vi "RemoteVI Index HTML.vi"(11 "error in":errorcluster) -> (4 "html":string, 15 "error out":errorcluster)   [LabVIEW 2020, in "RemoteVI.lvlib"]
doc: "Returns the browser client, web\\index.html, as one string constant (45029 bytes, SHA-256 bd4df0f21e4f24879766d9c2ba5b297a308cdc7323f2ba91d4f2f1fba401afc3). Generated by scripts\\gen-index-html-vi.mjs - do not edit the constant by hand; regenerate it when the client changes. error in passes through unchanged."
uses:
  RemoteVI.lvlib
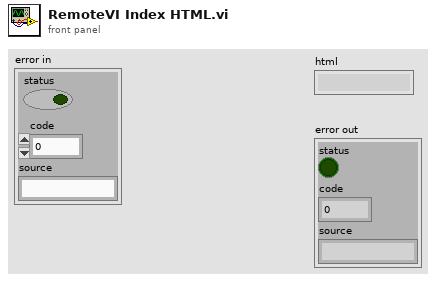
[diagram p1: front panel]
diagram:
  # "Generated from web/index.html"
  "html" <- "<!doctype html>\r\n<html lang=\"en\">\r\n<head>\r\n<meta charset=\"utf-8\">\r\n<meta name=\"viewport\" content=\"width=device-width, initial-scale=1, viewport-fit=cover\">\r\n<title>RemoteVI</title>\r\n<!--\r\n  RemoteVI browser client, protocol v2 (docs/protocol.md).\r\n  Self-contained on purpose: the LabVIEW toolkit embeds this one file as a string\r\n  constant and serves it for GET /, so a built EXE needs no support files.\r\n  Keep it pure ASCII (use \\u escapes and HTML entities) so the G string constant\r\n  holds exactly these bytes. After editing, regenerate the embedded copy:\r\n  node scripts/gen-index-html-vi.mjs --compose\r\n-->\r\n<style>\r\n:root {\r\n  --bg: #e9ebee; --bar-bg: #fff; --bar-fg: #1d2330; --muted: #667085;\r\n  --accent: #1f6feb; --ok: #1a7f37; --warn: #bf8700; --err: #cf222e; --border: #d0d7de;\r\n  --btn-hover: rgb(0 0 0 / 0.06);\r\n  color-scheme: light dark;\r\n}\r\n@media (prefers-color-scheme: dark) {\r\n  :root { --bg: #15181e; --bar-bg: #1e232b; --bar-fg: #e6edf3; --muted: #8d96a0; --border: #30363d; --btn-hover: rgb(255 255 255 / 0.08); }\r\n}\r\n* { box-sizing: border-box; }\r\nhtml, body { height: 100%; margin: 0; }\r\nbody {\r\n  display: flex; flex-direction: column; background: var(--bg); color: var(--bar-fg);\r\n  font: 13px/1.4 system-ui, -apple-system, \"Segoe UI\", sans-serif;\r\n}\r\n.bar {\r\n  display: flex; align-items: center; gap: 8px; padding: 6px 12px;\r\n  padding-left: max(12px, env(safe-area-inset-left)); padding-right: max(12px, env(safe-area-inset-right));\r\n  background: var(--bar-bg); border-bottom: 1px solid var(--border); flex-wrap: nowrap; min-height: 40px;\r\n}\r\n.title { display: flex; align-items: center; gap: 8px; min-width: 0; }\r\n.title strong { white-space: nowrap; overflow: hidden; text-overflow: ellipsis; }\r\n#status { color: var(--muted); white-space: nowrap; }\r\n.spacer { flex: 1; }\r\n.stats { color: var(--muted); font-variant-numeric: tabular-nums; white-space: nowrap; }\r\n.group { display: inline-flex; border: 1px solid var(--border); border-radius: 6px; overflow: hidden; }\r\n.group button + button { border-left: 1px solid var(--border); }\r\n.bar button {\r\n  font: inherit; min-width: 32px; height: 28px; padding: 0 9px; border: 0; background: transparent;\r\n  color: inherit; cursor: pointer; white-space: nowrap;\r\n}\r\n.bar > button { border: 1px solid var(--border); border-radius: 6px; }\r\n.bar button:hover { background: var(--btn-hover); }\r\n.bar button[aria-pressed=\"true\"] { color: var(--accent); background: color-mix(in srgb, var(--accent) 12%, transparent); }\r\n#zoom-label { min-width: 48px; text-align: center; color: var(--muted); font-variant-numeric: tabular-nums; }\r\n.dot { width: 9px; height: 9px; flex: none; border-radius: 50%; background: var(--warn); }\r\nbody[data-state=\"online\"] .dot { background: var(--ok); }\r\nbody[data-state=\"offline\"] .dot { background: var(--err); }\r\n#kbd-btn { display: none; }\r\nbody[data-touch=\"true\"] #kbd-btn { display: inline-block; }\r\n\r\n/* The stage scrolls; the wrapper is sized to the scaled frame so scrollbars match. */\r\n.stage { flex: 1; overflow: auto; padding: 16px; overscroll-behavior: contain; }\r\n.panel-wrap {\r\n  position: relative; margin: 0 auto; box-shadow: 0 1px 6px rgb(0 0 0 / 0.25);\r\n  touch-action: none; transform-origin: 0 0;\r\n}\r\n#panel { display: block; outline: none; cursor: default; touch-action: none; }\r\n#panel.pixelated { image-rendering: pixelated; }\r\nbody[data-view-only=\"true\"] #panel { cursor: not-allowed; }\r\n/* LabVIEW popups (menus, dropdowns, palette popups); may extend past the panel. */\r\n#overlay { position: absolute; left: 0; top: 0; transform-origin: 0 0; pointer-events: none; }\r\n#overlay img { position: absolute; display: block; pointer-events: auto; box-shadow: 2px 2px 6px rgb(0 0 0 / 0.35); }\r\n#overlay.pixelated img { image-rendering: pixelated; }\r\n/* Other windows of the application (dialogs, file dialogs, subVI panels). */\r\n#windows { position: absolute; left: 0; top: 0; width: 0; height: 0; }\r\n.win {\r\n  position: absolute; display: flex; flex-direction: column; background: var(--bar-bg);\r\n  border: 1px solid var(--border); border-radius: 8px; overflow: hidden;\r\n  box-shadow: 0 8px 28px rgb(0 0 0 / 0.35), 0 1px 4px rgb(0 0 0 / 0.2);\r\n}\r\n.win.active { border-color: var(--accent); }\r\n.win-title {\r\n  display: flex; align-items: center; gap: 8px; height: 30px; padding: 0 6px 0 10px; flex: none;\r\n  font-weight: 600; cursor: move; user-select: none; touch-action: none; border-bottom: 1px solid var(--border);\r\n}\r\n.win.active .win-title { background: color-mix(in srgb, var(--accent) 10%, var(--bar-bg)); }\r\n.win-title span { flex: 1; overflow: hidden; text-overflow: ellipsis; white-space: nowrap; }\r\n.win-title button {\r\n  width: 26px; height: 22px; border: 0; border-radius: 4px; background: transparent; color: inherit; font: inherit; cursor: pointer;\r\n}\r\n.win-title button:hover { background: var(--err); color: #fff; }\r\n.win canvas { display: block; touch-action: none; }\r\n.win canvas.pixelated { image-rendering: pixelated; }\r\n/* While a modal window is up the panel is disabled, as on the host. */\r\n#dim { position: absolute; inset: 0; background: rgb(0 0 0 / 0.28); display: none; }\r\n.panel-wrap.modal #dim { display: block; }\r\n#win-list { max-width: 180px; height: 28px; font: inherit; border: 1px solid var(--border); border-radius: 6px; background: var(--bar-bg); color: inherit; }\r\n#win-list[hidden] { display: none; }\r\n/* Tip strip of the control under the pointer, drawn like LabVIEW's own (tips message). */\r\n#tip {\r\n  position: fixed; z-index: 1000; display: none; max-width: 400px; padding: 2px 5px;\r\n  background: #ffffe1; color: #000; border: 1px solid #767676; box-shadow: 1px 2px 4px rgb(0 0 0 / 0.3);\r\n  font: 12px/1.35 \"Segoe UI\", Tahoma, sans-serif; white-space: pre-wrap; pointer-events: none;\r\n}\r\n#tip.show { display: block; }\r\n/* Splitter bars (splitters message): the client drags them itself and shows this line meanwhile. */\r\n#ghost { position: absolute; display: none; pointer-events: none; background: rgb(0 0 0 / 0.45); outline: 1px dashed #fff; }\r\n#ghost.show { display: block; }\r\n.panel-wrap.split-v, .panel-wrap.split-v #panel { cursor: col-resize; }\r\n.panel-wrap.split-h, .panel-wrap.split-h #panel { cursor: row-resize; }\r\n/* Hidden input that brings up the on-screen keyboard on touch devices. */\r\n#kbd { position: fixed; left: 0; bottom: 0; width: 1px; height: 1px; opacity: 0; border: 0; padding: 0; font-size: 16px; }\r\n.toast {\r\n  position: fixed; left: 50%; bottom: 24px; transform: translateX(-50%); padding: 6px 12px; border-radius: 6px;\r\n  background: rgb(0 0 0 / 0.75); color: #fff; font-size: 12px; pointer-events: none; opacity: 0; transition: opacity 0.3s;\r\n}\r\n.toast.show { opacity: 1; }\r\n@media (max-width: 720px) {\r\n  .stats, #status, #zoom-label { display: none; }\r\n  .bar { gap: 6px; padding-top: 4px; padding-bottom: 4px; }\r\n  .stage { padding: 8px; }\r\n}\r\n</style>\r\n</head>\r\n<body data-state=\"connecting\" data-touch=\"false\">\r\n<header class=\"bar\">\r\n  <span class=\"title\"><span class=\"dot\" aria-hidden=\"true\"></span><strong id=\"vi-name\">RemoteVI</strong></span>\r\n  <span id=\"status\" role=\"status\">Connecting&hellip;</span>\r\n  <span class=\"spacer\"></span>\r\n  <span id=\"stats\" class=\"stats\"></span>\r\n  <span class=\"group\" role=\"group\" aria-label=\"Scaling\">\r\n    <button type=\"button\" data-mode=\"actual\" title=\"Actual size: one LabVIEW pixel per screen pixel (1)\">1:1</button>\r\n    <button type=\"button\" data-mode=\"fit\" title=\"Fit the whole window into the view (F)\">Fit</button>\r\n    <button type=\"button\" data-mode=\"width\" title=\"Fit the width, scroll vertically (W)\">Width</button>\r\n  </span>\r\n  <span class=\"group\" role=\"group\" aria-label=\"Zoom\">\r\n    <button type=\"button\" id=\"zoom-out\" title=\"Zoom out (-)\">&minus;</button>\r\n    <button type=\"button\" id=\"zoom-label\" title=\"Back to actual size\">100%</button>\r\n    <button type=\"button\" id=\"zoom-in\" title=\"Zoom in (+)\">+</button>\r\n  </span>\r\n  <select id=\"win-list\" title=\"Open windows\" hidden></select>\r\n  <button type=\"button\" id=\"kbd-btn\" title=\"Show the on-screen keyboard\">&#x2328;</button>\r\n  <button type=\"button\" id=\"fs-btn\" title=\"Fullscreen\">&#x26F6;</button>\r\n</header>\r\n<main id=\"stage\" class=\"stage\">\r\n  <div class=\"panel-wrap\" id=\"wrap\">\r\n    <canvas id=\"panel\" tabindex=\"0\" width=\"1\" height=\"1\" aria-label=\"Remote front panel\"></canvas>\r\n    <div id=\"dim\"></div>\r\n    <div id=\"windows\"></div>\r\n    <div id=\"overlay\"></div>\r\n    <div id=\"ghost\"></div>\r\n  </div>\r\n</main>\r\n<input id=\"kbd\" type=\"text\" autocomplete=\"off\" autocapitalize=\"off\" autocorrect=\"off\" spellcheck=\"false\" aria-label=\"Keyboard input\">\r\n<div id=\"toast\" class=\"toast\" role=\"status\"></div>\r\n<div id=\"tip\" role=\"tooltip\"></div>\r\n<script>\r\n'use strict';\r\n\r\n// --- protocol v2 constants (docs/protocol.md) --------------------------------\r\n\r\nconst FRAME_MAGIC = 0x52;          // 'R'\r\nconst MSG_FRAME = 1;\r\nconst MSG_OVERLAY = 2;\r\nconst MSG_WINDOW_FRAME = 3;\r\nconst OVERLAY_HEADER = 4;          // magic, type, count u16\r\nconst WINDOW_FRAME_HEADER = 16;    // magic, type, id u32, seq u32, width u16, height u16, count u16\r\nconst WIN_TITLE_H = 31;            // CSS px of a window's title bar (+ border)\r\nconst FRAME_HEADER = 12;           // magic, type, seq u32, width u16, height u16, count u16\r\nconst RECT_HEADER = 8;             // x i16, y i16, length u32\r\n\r\n// Win32 message numbers. The server posts them to the panel window, so these\r\n// values ARE the protocol.\r\nconst WM = {\r\n  KEYDOWN: 0x0100, KEYUP: 0x0101, CHAR: 0x0102,\r\n  MOUSEMOVE: 0x0200,\r\n  LBUTTONDOWN: 0x0201, LBUTTONUP: 0x0202, LBUTTONDBLCLK: 0x0203,\r\n  RBUTTONDOWN: 0x0204, RBUTTONUP: 0x0205, RBUTTONDBLCLK: 0x0206,\r\n  MBUTTONDOWN: 0x0207, MBUTTONUP: 0x0208, MBUTTONDBLCLK: 0x0209,\r\n  MOUSEWHEEL: 0x020A,\r\n};\r\nconst MK = { LBUTTON: 0x01, RBUTTON: 0x02, SHIFT: 0x04, CONTROL: 0x08, MBUTTON: 0x10 };\r\nconst WHEEL_DELTA = 120;\r\n\r\n// Browser button index (0 left, 1 middle, 2 right) -> [down, up, dblclk].\r\nconst BUTTON_MSGS = {\r\n  0: [WM.LBUTTONDOWN, WM.LBUTTONUP, WM.LBUTTONDBLCLK],\r\n  1: [WM.MBUTTONDOWN, WM.MBUTTONUP, WM.MBUTTONDBLCLK],\r\n  2: [WM.RBUTTONDOWN, WM.RBUTTONUP, WM.RBUTTONDBLCLK],\r\n};\r\n\r\n// KeyboardEvent.code -> [virtual-key code, extended-key flag]. Printable\r\n// characters are not listed: they travel as WM_CHAR so the remote side does not\r\n// depend on the host's keyboard layout.\r\nconst VK = {\r\n  Backspace: [0x08, 0], Tab: [0x09, 0], Enter: [0x0D, 0], NumpadEnter: [0x0D, 1],\r\n  ShiftLeft: [0x10, 0], ShiftRight: [0x10, 0], ControlLeft: [0x11, 0], ControlRight: [0x11, 1],\r\n  Escape: [0x1B, 0], PageUp: [0x21, 1], PageDown: [0x22, 1], End: [0x23, 1], Home: [0x24, 1],\r\n  ArrowLeft: [0x25, 1], ArrowUp: [0x26, 1], ArrowRight: [0x27, 1], ArrowDown: [0x28, 1],\r\n  Insert: [0x2D, 1], Delete: [0x2E, 1],\r\n  F1: [0x70, 0], F2: [0x71, 0], F3: [0x72, 0], F4: [0x73, 0], F5: [0x74, 0], F6: [0x75, 0],\r\n  F7: [0x76, 0], F8: [0x77, 0], F9: [0x78, 0], F10: [0x79, 0], F11: [0x7A, 0], F12: [0x7B, 0],\r\n};\r\n\r\nconst ZOOM_STEPS = [0.25, 0.33, 0.5, 0.67, 0.75, 0.9, 1, 1.25, 1.5, 2, 2.5, 3, 4];\r\nconst ZOOM_MIN = 0.1;\r\nconst ZOOM_MAX = 4;\r\nconst LONG_PRESS_MS = 550;      // touch: hold this long without moving = right click\r\nconst TAP_SLOP_PX = 8;          // touch: moving further than this starts a drag\r\nconst TIP_DELAY_MS = 500;       // hover this long on a control to see its tip strip\r\n\r\nfunction mouseFlags(e) {\r\n  let w = 0;\r\n  if (e.buttons & 1) w |= MK.LBUTTON;\r\n  if (e.buttons & 2) w |= MK.RBUTTON;\r\n  if (e.buttons & 4) w |= MK.MBUTTON;\r\n  if (e.shiftKey) w |= MK.SHIFT;\r\n  if (e.ctrlKey) w |= MK.CONTROL;\r\n  return w;\r\n}\r\n\r\n// lParam for WM_KEYDOWN / WM_KEYUP: repeat count 1, extended bit 24, and for\r\n// key-up the previous-state and transition bits. Sent as an unsigned decimal.\r\nfunction keyLParam(extended, up) {\r\n  let l = 1;\r\n  if (extended) l += 0x01000000;\r\n  if (up) l += 0xC0000000;\r\n  return l;\r\n}\r\n\r\nfunction readRects(v, buf, o, count) {\r\n  const rects = [];\r\n  for (let i = 0; i < count; i++) {\r\n    if (o + RECT_HEADER > buf.byteLength) throw new Error('truncated message');\r\n    const x = v.getInt16(o), y = v.getInt16(o + 2), len = v.getUint32(o + 4);\r\n    o += RECT_HEADER;\r\n    if (o + len > buf.byteLength) throw new Error('truncated message');\r\n    rects.push({ x, y, png: new Blob([new Uint8Array(buf, o, len)], { type: 'image/png' }) });\r\n    o += len;\r\n  }\r\n  return rects;\r\n}\r\n\r\nfunction decodeOverlay(buf) {\r\n  const v = new DataView(buf);\r\n  return readRects(v, buf, OVERLAY_HEADER, v.getUint16(2));\r\n}\r\n\r\nfunction decodeWindowFrame(buf) {\r\n  const v = new DataView(buf);\r\n  if (buf.byteLength < WINDOW_FRAME_HEADER) throw new Error('truncated window frame');\r\n  return {\r\n    id: v.getUint32(2), seq: v.getUint32(6), width: v.getUint16(10), height: v.getUint16(12),\r\n    rects: readRects(v, buf, WINDOW_FRAME_HEADER, v.getUint16(14)),\r\n  };\r\n}\r\n\r\nfunction decodeFrame(buf) {\r\n  const v = new DataView(buf);\r\n  if (buf.byteLength < FRAME_HEADER || v.getUint8(0) !== FRAME_MAGIC || v.getUint8(1) !== MSG_FRAME) {\r\n    throw new Error('not a RemoteVI frame');\r\n  }\r\n  return {\r\n    seq: v.getUint32(2), width: v.getUint16(6), height: v.getUint16(8),\r\n    rects: readRects(v, buf, FRAME_HEADER, v.getUint16(10)),\r\n  };\r\n}\r\n\r\n// Per-viewer preference; storage can be unavailable (private mode, blocked site data).\r\nconst prefs = {\r\n  get(key, fallback) {\r\n    try { return localStorage.getItem(`remotevi.${key}`) ?? fallback; } catch { return fallback; }\r\n  },\r\n  set(key, value) {\r\n    try { localStorage.setItem(`remotevi.${key}`, value); } catch { /* not persisted */ }\r\n  },\r\n};\r\n\r\n// --- client -------------------------------------------------------------------\r\n\r\nclass RemoteViClient {\r\n  constructor() {\r\n    this.canvas = document.getElementById('panel');\r\n    this.wrap = document.getElementById('wrap');\r\n    this.overlay = document.getElementById('overlay');\r\n    this.ctx = this.canvas.getContext('2d', { alpha: false });\r\n    this.stage = document.getElementById('stage');\r\n    this.statusEl = document.getElementById('status');\r\n    this.statsEl = document.getElementById('stats');\r\n    this.kbd = document.getElementById('kbd');\r\n    this.ws = null;\r\n    this.backoff = 250;\r\n    this.queue = Promise.resolve();   // frames are painted strictly in order\r\n    this.pendingMove = null;\r\n    this.stats = { frames: 0, bytes: 0, since: performance.now() };\r\n    this.origin = { x: 0, y: 0 };     // where the panel starts inside the frame\r\n    this.touches = new Map();         // pointerId -> {x, y} for touch gestures\r\n    this.touch = null;                // single-finger state (tap / long press / drag)\r\n    this.pinch = null;                // two-finger state\r\n    this.windows = new Map();         // id -> {info, el, canvas, ctx, dx, dy} (docs/protocol.md 7)\r\n    this.windowsLayer = document.getElementById('windows');\r\n    this.winList = document.getElementById('win-list');\r\n    this.pressWin = null;             // window a mouse press started in (keeps a drag on it)\r\n    this.tips = [];                   // tip strips {x, y, w, h, text} in frame coordinates (tips message)\r\n    this.tipEl = document.getElementById('tip');\r\n    this.tip = { at: null, timer: 0, quiet: null };  // control hovered, dwell timer, tip silenced by a click\r\n    this.splitters = [];              // draggable splitter bars {id, x, y, w, h, vertical, min, max} (splitters message)\r\n    this.split = null;                // splitter drag in progress {bar, pos, pointerId}\r\n    this.ghost = document.getElementById('ghost');\r\n\r\n    const coarse = matchMedia('(pointer: coarse)').matches;\r\n    document.body.dataset.touch = String(coarse);\r\n    this.mode = prefs.get('mode', coarse ? 'width' : 'actual');\r\n    this.zoom = Number(prefs.get('zoom', '1')) || 1;\r\n\r\n    this.bindView();\r\n    this.bindInput();\r\n    this.bindKeyboard();\r\n    this.winList.addEventListener('change', () => {\r\n      const w = this.windows.get(Number(this.winList.value));\r\n      if (w) { this.raise(w); w.el.scrollIntoView({ block: 'nearest', inline: 'nearest' }); }\r\n    });\r\n    setInterval(() => this.showStats(), 1000);\r\n    this.applyView();\r\n    this.connect();\r\n  }\r\n\r\n  // --- connection ----------------------------------------------------------------\r\n\r\n  connect() {\r\n    const scheme = location.protocol === 'https:' ? 'wss' : 'ws';\r\n    // The share's access token travels in the page URL (?t=...) and is required for the WebSocket too.\r\n    const token = new URLSearchParams(location.search).get('t') ?? '';\r\n    const ws = new WebSocket(`${scheme}://${location.host}/ws?t=${encodeURIComponent(token)}`);\r\n    ws.binaryType = 'arraybuffer';\r\n    this.ws = ws;\r\n    this.setStatus('connecting', 'Connecting...');\r\n    let opened = false;\r\n    ws.onopen = () => { opened = true; this.backoff = 250; this.setStatus('online', 'Connected'); };\r\n    ws.onmessage = (ev) => {\r\n      if (typeof ev.data === 'string') this.onText(ev.data);\r\n      else this.onFrame(ev.data);\r\n    };\r\n    ws.onclose = () => {\r\n      if (this.ws !== ws) return;\r\n      const retry = `retrying in ${(this.backoff / 1000).toFixed(1)} s`;\r\n      // The server answers a missing or wrong token with 403, which a browser reports as a plain close.\r\n      const why = opened ? 'Disconnected'\r\n        : !token ? 'This link has no access token (?t=...): open the full link of the share'\r\n          : 'Not connected: the access token is wrong, or the share has stopped';\r\n      this.setStatus('offline', `${why}, ${retry}`);\r\n      setTimeout(() => this.connect(), this.backoff);\r\n      this.backoff = Math.min(this.backoff * 2, 5000);\r\n    };\r\n  }\r\n\r\n  send(line) {\r\n    if (this.ws?.readyState === WebSocket.OPEN) this.ws.send(line);\r\n  }\r\n\r\n  onText(text) {\r\n    // Server text messages (docs/protocol.md 3.3). Unknown ones are ignored.\r\n    const sp = text.indexOf(' ');\r\n    const cmd = sp < 0 ? text : text.slice(0, sp);\r\n    const arg = sp < 0 ? '' : text.slice(sp + 1);\r\n    if (cmd === 'title') {\r\n      document.getElementById('vi-name').textContent = arg;\r\n      document.title = `${arg} - RemoteVI`;\r\n    } else if (cmd === 'viewonly') {\r\n      document.body.dataset.viewOnly = String(arg === '1');\r\n    } else if (cmd === 'windows') {\r\n      let list;\r\n      try { list = JSON.parse(arg); } catch { return; }\r\n      if (Array.isArray(list)) this.updateWindows(list);\r\n    } else if (cmd === 'origin') {\r\n      const [x, y] = arg.split(' ').map(Number);\r\n      if (Number.isFinite(x) && Number.isFinite(y)) this.origin = { x, y };\r\n    } else if (cmd === 'tips') {\r\n      let list;\r\n      try { list = JSON.parse(arg); } catch { return; }\r\n      if (!Array.isArray(list)) return;\r\n      this.tips = list.filter((t) => t && typeof t.text === 'string'\r\n        && [t.x, t.y, t.w, t.h].every(Number.isFinite));\r\n      this.hideTip();\r\n    } else if (cmd === 'splitters') {\r\n      let list;\r\n      try { list = JSON.parse(arg); } catch { return; }\r\n      if (!Array.isArray(list)) return;\r\n      this.splitters = list.filter((b) => b && Number.isInteger(b.id)\r\n        && [b.x, b.y, b.w, b.h, b.min, b.max].every(Number.isFinite));\r\n    }\r\n  }\r\n\r\n  // --- splitter bars (docs/protocol.md 3.3, 4) ----------------------------------------\r\n  // LabVIEW moves a splitter bar only while it tracks the real mouse, so the client drags\r\n  // the bar itself (a line follows the pointer) and sends `s <id> <pos>` on release; the\r\n  // server sets the splitter's position through VI Server.\r\n\r\n  /** The draggable bar under a client point, or null (not over a popup, a window or while modal). */\r\n  splitterAt(clientX, clientY) {\r\n    if (!this.splitters.length || this.overlay.childElementCount || this.wrap.classList.contains('modal')\r\n        || this.windowAt(clientX, clientY)) return null;\r\n    const { x, y } = this.framePoint(clientX, clientY, null);\r\n    // A thin bar is easier to hit with a few pixels of slack across it.\r\n    return this.splitters.find((b) => {\r\n      const sx = b.vertical ? 3 : 0, sy = b.vertical ? 0 : 3;\r\n      return x >= b.x - sx && x < b.x + b.w + sx && y >= b.y - sy && y < b.y + b.h + sy;\r\n    }) ?? null;\r\n  }\r\n\r\n  /** Cursor hint over a bar. */\r\n  splitterHover(clientX, clientY) {\r\n    const b = this.split?.bar ?? this.splitterAt(clientX, clientY);\r\n    this.wrap.classList.toggle('split-v', !!b?.vertical);\r\n    this.wrap.classList.toggle('split-h', !!b && !b.vertical);\r\n  }\r\n\r\n  splitStart(bar, e) {\r\n    this.hideTip(true);\r\n    this.split = { bar, pos: bar.vertical ? bar.x : bar.y, pointerId: e.pointerId, moved: false };\r\n    this.wrap.setPointerCapture(e.pointerId);\r\n    this.splitMove(e);\r\n  }\r\n\r\n  splitMove(e) {\r\n    const s = this.split;\r\n    const b = s.bar;\r\n    const { x, y } = this.framePoint(e.clientX, e.clientY, null);\r\n    const at = Math.round((b.vertical ? x - b.w / 2 : y - b.h / 2));\r\n    const pos = Math.max(b.min, Math.min(b.max, at));\r\n    if (pos !== s.pos) s.moved = true;\r\n    s.pos = pos;\r\n    const z = this.zoom;\r\n    const g = this.ghost.style;\r\n    g.left = `${(b.vertical ? pos : b.x) * z}px`;\r\n    g.top = `${(b.vertical ? b.y : pos) * z}px`;\r\n    g.width = `${Math.max(2, b.w * z)}px`;\r\n    g.height = `${Math.max(2, b.h * z)}px`;\r\n    this.ghost.classList.add('show');\r\n  }\r\n\r\n  splitEnd(cancel) {\r\n    const s = this.split;\r\n    this.split = null;\r\n    this.ghost.classList.remove('show');\r\n    if (!s || cancel || !s.moved) return;\r\n    const b = s.bar;\r\n    this.send(`s ${b.id} ${s.pos}`);\r\n  }\r\n\r\n  // --- tip strips (docs/protocol.md 3.3) ----------------------------------------------\r\n  // LabVIEW shows tip strips only while it is the foreground application, so the\r\n  // server sends the texts and the client shows them itself after a hover dwell.\r\n\r\n  /** Pointer at a client point (mouse, no button held): start, keep or hide the tip. */\r\n  hoverTip(clientX, clientY) {\r\n    let hit = null;\r\n    if (!this.overlay.childElementCount && !this.wrap.classList.contains('modal')\r\n        && !this.windowAt(clientX, clientY)) {\r\n      const { x, y } = this.framePoint(clientX, clientY, null);\r\n      hit = this.tips.find((t) => x >= t.x && y >= t.y && x < t.x + t.w && y < t.y + t.h) ?? null;\r\n    }\r\n    this.tip.pos = { x: clientX, y: clientY };\r\n    if (hit === this.tip.at) return;\r\n    this.hideTip();\r\n    this.tip.at = hit;\r\n    if (this.tip.quiet && hit !== this.tip.quiet) this.tip.quiet = null;\r\n    if (hit && hit !== this.tip.quiet) this.tip.timer = setTimeout(() => this.showTip(hit), TIP_DELAY_MS);\r\n  }\r\n\r\n  showTip(t) {\r\n    const el = this.tipEl;\r\n    el.textContent = t.text;\r\n    el.classList.add('show');\r\n    // Below and right of the pointer, as Windows places tooltips; kept inside the view.\r\n    const { x, y } = this.tip.pos;\r\n    const r = el.getBoundingClientRect();\r\n    el.style.left = `${Math.max(0, Math.min(x + 2, innerWidth - r.width - 2))}px`;\r\n    el.style.top = `${y + 22 + r.height > innerHeight ? Math.max(0, y - r.height - 4) : y + 22}px`;\r\n  }\r\n\r\n  /** Hide the tip; with silence, it stays hidden until the pointer leaves that control (a click). */\r\n  hideTip(silence = false) {\r\n    clearTimeout(this.tip.timer);\r\n    if (silence && this.tip.at) this.tip.quiet = this.tip.at;\r\n    if (!silence) this.tip.at = null;\r\n    this.tipEl.classList.remove('show');\r\n  }\r\n\r\n  onFrame(buf) {\r\n    if (buf.byteLength >= 2 && new DataView(buf).getUint8(1) === MSG_WINDOW_FRAME) {\r\n      let wf;\r\n      try { wf = decodeWindowFrame(buf); } catch (err) { console.error(err); return; }\r\n      this.stats.bytes += buf.byteLength;\r\n      this.queue = this.queue.then(() => this.paintWindow(wf)).catch((err) => console.error(err));\r\n      return;\r\n    }\r\n    if (buf.byteLength >= 2 && new DataView(buf).getUint8(1) === MSG_OVERLAY) {\r\n      let popups;\r\n      try { popups = decodeOverlay(buf); } catch (err) { console.error(err); return; }\r\n      this.queue = this.queue.then(() => this.showOverlay(popups));\r\n      return;\r\n    }\r\n    let frame;\r\n    try {\r\n      frame = decodeFrame(buf);\r\n    } catch (err) {\r\n      console.error(err);\r\n      return;\r\n    }\r\n    this.stats.frames++;\r\n    this.stats.bytes += buf.byteLength;\r\n    this.queue = this.queue.then(() => this.paint(frame)).catch((err) => console.error(err));\r\n  }\r\n\r\n  async paint(frame) {\r\n    const bitmaps = await Promise.all(frame.rects.map((r) => createImageBitmap(r.png)));\r\n    if (frame.width !== this.canvas.width || frame.height !== this.canvas.height) {\r\n      this.canvas.width = frame.width;\r\n      this.canvas.height = frame.height;\r\n      this.applyView();\r\n    }\r\n    frame.rects.forEach((r, i) => {\r\n      this.ctx.drawImage(bitmaps[i], r.x, r.y);\r\n      bitmaps[i].close();\r\n    });\r\n    // Ack after painting: the server keeps at most two frames in flight, so a\r\n    // slow client gets fresher frames instead of a growing backlog.\r\n    this.send(`a ${frame.seq}`);\r\n  }\r\n\r\n  showOverlay(popups) {\r\n    if (popups.length) this.hideTip(true);\r\n    for (const img of this.overlay.querySelectorAll('img')) URL.revokeObjectURL(img.src);\r\n    this.overlay.replaceChildren(...popups.map((p) => {\r\n      const img = document.createElement('img');\r\n      img.src = URL.createObjectURL(p.png);\r\n      img.style.left = `${p.x}px`;\r\n      img.style.top = `${p.y}px`;\r\n      img.draggable = false;\r\n      return img;\r\n    }));\r\n  }\r\n\r\n  // --- other windows (docs/protocol.md 7) ------------------------------------------\r\n\r\n  updateWindows(list) {\r\n    const seen = new Set();\r\n    list.forEach((info, i) => {\r\n      seen.add(info.id);\r\n      let w = this.windows.get(info.id);\r\n      if (!w) {\r\n        w = this.createWindow(info);\r\n        this.windows.set(info.id, w);\r\n      }\r\n      w.info = info;\r\n      w.el.querySelector('.win-title span').textContent = info.title || 'Window';\r\n      w.el.querySelector('.win-title button').hidden = !info.closable;\r\n      w.el.classList.toggle('active', !!info.active);\r\n      w.el.style.zIndex = String(100 + list.length - i); // the list is front-most first\r\n    });\r\n    for (const [id, w] of this.windows) {\r\n      if (!seen.has(id)) { w.el.remove(); this.windows.delete(id); }\r\n    }\r\n    this.wrap.classList.toggle('modal', list.some((w) => w.modal));\r\n    this.winList.hidden = list.length === 0;\r\n    this.winList.replaceChildren(...list.map((w) => new Option(w.title || 'Window', String(w.id))));\r\n    this.layoutWindows();\r\n  }\r\n\r\n  createWindow(info) {\r\n    const el = document.createElement('div');\r\n    el.className = 'win';\r\n    el.innerHTML = '<div class=\"win-title\"><span></span><button type=\"button\" title=\"Close\">&#x2715;</button></div>';\r\n    const canvas = document.createElement('canvas');\r\n    canvas.width = Math.max(1, info.w);\r\n    canvas.height = Math.max(1, info.h);\r\n    el.append(canvas);\r\n    const w = { info, el, canvas, ctx: canvas.getContext('2d', { alpha: false }), dx: 0, dy: 0 };\r\n    // Narrow screens: open the window centred in the visible area.\r\n    if (innerWidth < 720) {\r\n      const z = this.zoom, r = this.stage.getBoundingClientRect(), wr = this.wrap.getBoundingClientRect();\r\n      w.dx = ((r.left + r.width / 2 - wr.left) / z) - (info.x + info.w / 2);\r\n      w.dy = ((r.top + r.height / 2 - wr.top) / z) - (info.y + info.h / 2);\r\n    }\r\n    const title = el.querySelector('.win-title');\r\n    title.querySelector('button').addEventListener('click', (e) => {\r\n      e.stopPropagation();\r\n      this.send(`x ${w.info.id}`);\r\n    });\r\n    title.addEventListener('pointerdown', (e) => {\r\n      e.stopPropagation();\r\n      if (e.target.closest('button')) return;\r\n      e.preventDefault();\r\n      this.raise(w);\r\n      try { title.setPointerCapture(e.pointerId); } catch { /* ignore */ }\r\n      const start = { x: e.clientX, y: e.clientY, dx: w.dx, dy: w.dy };\r\n      const move = (ev) => {\r\n        w.dx = start.dx + (ev.clientX - start.x) / this.zoom;\r\n        w.dy = start.dy + (ev.clientY - start.y) / this.zoom;\r\n        this.layoutWindows();\r\n      };\r\n      const end = () => {\r\n        title.removeEventListener('pointermove', move);\r\n        title.removeEventListener('pointerup', end);\r\n      };\r\n      title.addEventListener('pointermove', move);\r\n      title.addEventListener('pointerup', end);\r\n    });\r\n    for (const t of ['pointermove', 'pointerup', 'wheel', 'contextmenu']) title.addEventListener(t, (e) => e.stopPropagation());\r\n    this.windowsLayer.append(el);\r\n    return w;\r\n  }\r\n\r\n  raise(w) {\r\n    let top = 100;\r\n    for (const o of this.windows.values()) top = Math.max(top, Number(o.el.style.zIndex) || 0);\r\n    w.el.style.zIndex = String(top + 1);\r\n  }\r\n\r\n  layoutWindows() {\r\n    const z = this.zoom;\r\n    const crisp = Math.abs(z - Math.round(z)) < 0.001 && z >= 1;\r\n    for (const w of this.windows.values()) {\r\n      const { x, y } = w.info;\r\n      w.el.style.left = `${(x + w.dx) * z}px`;\r\n      w.el.style.top = `${(y + w.dy) * z - WIN_TITLE_H}px`;\r\n      w.canvas.style.width = `${w.canvas.width * z}px`;\r\n      w.canvas.style.height = `${w.canvas.height * z}px`;\r\n      w.canvas.classList.toggle('pixelated', crisp);\r\n    }\r\n  }\r\n\r\n  async paintWindow(f) {\r\n    const w = this.windows.get(f.id);\r\n    const bitmaps = await Promise.all(f.rects.map((r) => createImageBitmap(r.png)));\r\n    if (w) {\r\n      if (f.width !== w.canvas.width || f.height !== w.canvas.height) {\r\n        w.canvas.width = f.width;\r\n        w.canvas.height = f.height;\r\n        this.layoutWindows();\r\n      }\r\n      f.rects.forEach((r, i) => w.ctx.drawImage(bitmaps[i], r.x, r.y));\r\n    }\r\n    bitmaps.forEach((b) => b.close());\r\n    this.send(`a ${f.seq}`);\r\n  }\r\n\r\n  /** The window whose picture (not title bar) contains the client point, front-most first. */\r\n  windowAt(clientX, clientY) {\r\n    let best = null;\r\n    for (const w of this.windows.values()) {\r\n      const r = w.canvas.getBoundingClientRect();\r\n      if (clientX >= r.left && clientX < r.right && clientY >= r.top && clientY < r.bottom) {\r\n        if (!best || Number(w.el.style.zIndex) > Number(best.el.style.zIndex)) best = w;\r\n      }\r\n    }\r\n    return best;\r\n  }\r\n\r\n  // --- view: scaling modes, zoom, fullscreen -------------------------------------\r\n\r\n  bindView() {\r\n    for (const b of document.querySelectorAll('[data-mode]')) {\r\n      b.addEventListener('click', () => this.setMode(b.dataset.mode));\r\n    }\r\n    document.getElementById('zoom-in').addEventListener('click', () => this.stepZoom(1));\r\n    document.getElementById('zoom-out').addEventListener('click', () => this.stepZoom(-1));\r\n    document.getElementById('zoom-label').addEventListener('click', () => this.setMode('actual'));\r\n    const fs = document.getElementById('fs-btn');\r\n    if (!document.documentElement.requestFullscreen) fs.hidden = true;\r\n    fs.addEventListener('click', () => {\r\n      if (document.fullscreenElement) document.exitFullscreen();\r\n      else document.documentElement.requestFullscreen().catch(() => this.toast('Fullscreen not available'));\r\n    });\r\n    document.addEventListener('fullscreenchange', () => {\r\n      fs.setAttribute('aria-pressed', String(!!document.fullscreenElement));\r\n      this.applyView();\r\n    });\r\n    new ResizeObserver(() => this.applyView()).observe(this.stage);\r\n    // View shortcuts work when the panel does NOT have the keyboard focus.\r\n    document.addEventListener('keydown', (e) => {\r\n      if (document.activeElement === this.canvas || document.activeElement === this.kbd) return;\r\n      if (e.key === '1') this.setMode('actual');\r\n      else if (e.key === 'f' || e.key === 'F') this.setMode('fit');\r\n      else if (e.key === 'w' || e.key === 'W') this.setMode('width');\r\n      else if (e.key === '+' || e.key === '=') this.stepZoom(1);\r\n      else if (e.key === '-') this.stepZoom(-1);\r\n    });\r\n  }\r\n\r\n  setMode(mode) {\r\n    this.mode = mode;\r\n    if (mode === 'actual') this.zoom = 1;\r\n    prefs.set('mode', mode);\r\n    this.applyView();\r\n  }\r\n\r\n  stepZoom(dir) {\r\n    const z = this.zoom;\r\n    const next = dir > 0 ? ZOOM_STEPS.find((s) => s > z + 0.001) ?? ZOOM_MAX\r\n      : [...ZOOM_STEPS].reverse().find((s) => s < z - 0.001) ?? ZOOM_STEPS[0];\r\n    this.setZoom(next);\r\n  }\r\n\r\n  setZoom(z, anchor) {\r\n    const old = this.zoom;\r\n    this.zoom = Math.min(ZOOM_MAX, Math.max(ZOOM_MIN, z));\r\n    this.mode = this.zoom === 1 ? 'actual' : 'custom';\r\n    prefs.set('mode', this.mode);\r\n    prefs.set('zoom', String(this.zoom));\r\n    // Keep the point under the anchor (pinch midpoint) where it is.\r\n    let keep = null;\r\n    if (anchor) {\r\n      const r = this.wrap.getBoundingClientRect();\r\n      keep = { px: (anchor.x - r.left) / old, py: (anchor.y - r.top) / old, ax: anchor.x, ay: anchor.y };\r\n    }\r\n    this.applyView();\r\n    if (keep) {\r\n      const r = this.wrap.getBoundingClientRect();\r\n      this.stage.scrollLeft += r.left + keep.px * this.zoom - keep.ax;\r\n      this.stage.scrollTop += r.top + keep.py * this.zoom - keep.ay;\r\n    }\r\n  }\r\n\r\n  /** The zoom a mode implies for the current stage size. */\r\n  modeZoom() {\r\n    const w = this.canvas.width, h = this.canvas.height;\r\n    if (w <= 1 || h <= 1) return this.zoom;\r\n    const cs = getComputedStyle(this.stage);\r\n    const availW = this.stage.clientWidth - parseFloat(cs.paddingLeft) - parseFloat(cs.paddingRight);\r\n    const availH = this.stage.clientHeight - parseFloat(cs.paddingTop) - parseFloat(cs.paddingBottom);\r\n    if (this.mode === 'fit') return Math.max(ZOOM_MIN, Math.min(availW / w, availH / h));\r\n    if (this.mode === 'width') return Math.max(ZOOM_MIN, availW / w);\r\n    if (this.mode === 'actual') return 1;\r\n    return this.zoom;\r\n  }\r\n\r\n  applyView() {\r\n    if (this.mode !== 'custom') this.zoom = this.modeZoom();\r\n    const z = this.zoom;\r\n    const w = this.canvas.width, h = this.canvas.height;\r\n    this.canvas.style.width = `${w * z}px`;\r\n    this.canvas.style.height = `${h * z}px`;\r\n    // Pixel-exact at integer zoom; smooth when scaled down or by odd factors.\r\n    const crisp = Math.abs(z - Math.round(z)) < 0.001 && z >= 1;\r\n    this.canvas.classList.toggle('pixelated', crisp);\r\n    this.overlay.classList.toggle('pixelated', crisp);\r\n    this.overlay.style.transform = `scale(${z})`;\r\n    this.layoutWindows();\r\n    // Centre the frame when it is smaller than the stage (Fit), scroll when it is larger.\r\n    this.wrap.style.width = `${w * z}px`;\r\n    this.wrap.style.height = `${h * z}px`;\r\n    document.getElementById('zoom-label').textContent = `${Math.round(z * 100)}%`;\r\n    for (const b of document.querySelectorAll('[data-mode]')) {\r\n      b.setAttribute('aria-pressed', String(b.dataset.mode === this.mode));\r\n    }\r\n  }\r\n\r\n  // --- input -----------------------------------------------------------------------\r\n\r\n  // Frame pixel under a client point. Not clamped: popups may extend past the frame.\r\n  // A point over another window maps to host-layout coordinates (its x, y without the\r\n  // client-side drag offset), so the server always sees the layout of the host.\r\n  framePoint(clientX, clientY, win = this.windowAt(clientX, clientY)) {\r\n    if (win) {\r\n      const r = win.canvas.getBoundingClientRect();\r\n      return {\r\n        x: Math.floor((clientX - r.left) * (win.canvas.width / r.width)) + win.info.x,\r\n        y: Math.floor((clientY - r.top) * (win.canvas.height / r.height)) + win.info.y,\r\n      };\r\n    }\r\n    const r = this.canvas.getBoundingClientRect();\r\n    return {\r\n      x: Math.floor((clientX - r.left) * (this.canvas.width / r.width)),\r\n      y: Math.floor((clientY - r.top) * (this.canvas.height / r.height)),\r\n    };\r\n  }\r\n\r\n  mouseAt(msg, clientX, clientY, wParam) {\r\n    // A press keeps its window until the release, even when the pointer leaves it.\r\n    const win = this.pressWin ?? this.windowAt(clientX, clientY);\r\n    const { x, y } = this.framePoint(clientX, clientY, win);\r\n    this.send(`m ${msg} ${x} ${y} ${wParam >>> 0}`);\r\n  }\r\n\r\n  mouse(msg, e, wParam = mouseFlags(e)) {\r\n    this.mouseAt(msg, e.clientX, e.clientY, wParam);\r\n  }\r\n\r\n  bindInput() {\r\n    const c = this.canvas;\r\n    const w = this.wrap;\r\n    w.addEventListener('contextmenu', (e) => e.preventDefault());\r\n\r\n    w.addEventListener('pointerdown', (e) => {\r\n      if (this.split) return;\r\n      // A splitter bar is dragged by the client, by mouse or by one finger.\r\n      const bar = e.button === 0 && e.isPrimary && !(e.pointerType === 'touch' && this.touches.size)\r\n        ? this.splitterAt(e.clientX, e.clientY) : null;\r\n      if (bar && document.body.dataset.viewOnly !== 'true') { e.preventDefault(); this.splitStart(bar, e); return; }\r\n      if (e.pointerType === 'touch') { this.touchDown(e); return; }\r\n      const msgs = BUTTON_MSGS[e.button];\r\n      if (!msgs) return;\r\n      e.preventDefault();\r\n      this.hideTip(true);\r\n      c.focus({ preventScroll: true });\r\n      w.setPointerCapture(e.pointerId);\r\n      this.flushMove();\r\n      this.pressWin = this.windowAt(e.clientX, e.clientY);\r\n      if (this.pressWin) this.raise(this.pressWin);\r\n      // Windows reports the second press of a double click as *BUTTONDBLCLK.\r\n      this.mouse(e.detail === 2 ? msgs[2] : msgs[0], e);\r\n    });\r\n\r\n    const up = (e) => {\r\n      if (this.split?.pointerId === e.pointerId) { this.splitEnd(e.type === 'pointercancel'); this.splitterHover(e.clientX, e.clientY); return; }\r\n      if (e.pointerType === 'touch') { this.touchUp(e); return; }\r\n      const msgs = BUTTON_MSGS[e.button];\r\n      if (!msgs) return;\r\n      this.flushMove();\r\n      this.mouse(msgs[1], e);\r\n      this.pressWin = null;\r\n    };\r\n    w.addEventListener('pointerup', up);\r\n    w.addEventListener('pointercancel', up);\r\n\r\n    // Moves are coalesced to one per animation frame: only the latest position matters.\r\n    w.addEventListener('pointermove', (e) => {\r\n      if (this.split?.pointerId === e.pointerId) { this.splitMove(e); return; }\r\n      if (e.pointerType !== 'touch' && !e.buttons) this.splitterHover(e.clientX, e.clientY);\r\n      if (e.pointerType === 'touch') { this.touchMove(e); return; }\r\n      if (e.buttons) this.hideTip(true); else this.hoverTip(e.clientX, e.clientY);\r\n      const first = this.pendingMove === null;\r\n      this.pendingMove = e;\r\n      if (first) requestAnimationFrame(() => this.flushMove());\r\n    });\r\n\r\n    w.addEventListener('pointerleave', () => { this.hideTip(); this.tip.quiet = null; });\r\n\r\n    w.addEventListener('wheel', (e) => {\r\n      e.preventDefault();\r\n      this.hideTip(true);\r\n      if (e.ctrlKey) {\r\n        // Ctrl+wheel and trackpad pinch zoom the view, as in any browser page.\r\n        this.setZoom(this.zoom * (e.deltaY < 0 ? 1.1 : 1 / 1.1), { x: e.clientX, y: e.clientY });\r\n        return;\r\n      }\r\n      const notches = e.deltaMode === 0 ? -e.deltaY / 100 : -e.deltaY / 3;\r\n      const delta = Math.round(Math.max(-3, Math.min(3, notches || -Math.sign(e.deltaY))) * WHEEL_DELTA);\r\n      if (!delta) return;\r\n      // The wheel delta is the signed high word of wParam.\r\n      this.mouse(WM.MOUSEWHEEL, e, (delta & 0xFFFF) * 0x10000 + mouseFlags(e));\r\n    }, { passive: false });\r\n\r\n    c.addEventListener('keydown', (e) => this.keyDown(e));\r\n    c.addEventListener('keyup', (e) => this.keyUp(e));\r\n  }\r\n\r\n  flushMove() {\r\n    const e = this.pendingMove;\r\n    this.pendingMove = null;\r\n    if (e) this.mouse(WM.MOUSEMOVE, e);\r\n  }\r\n\r\n  // Touch: one finger is the mouse (tap = click, hold = right click, slide = drag);\r\n  // two fingers zoom and pan the view.\r\n  touchDown(e) {\r\n    e.preventDefault();\r\n    try { this.wrap.setPointerCapture(e.pointerId); } catch { /* pointer already gone */ }\r\n    this.touches.set(e.pointerId, { x: e.clientX, y: e.clientY });\r\n    if (this.touches.size === 2) {\r\n      this.cancelTouch();\r\n      const [a, b] = [...this.touches.values()];\r\n      this.pinch = {\r\n        dist: Math.hypot(a.x - b.x, a.y - b.y) || 1, zoom: this.zoom,\r\n        mid: { x: (a.x + b.x) / 2, y: (a.y + b.y) / 2 },\r\n      };\r\n      return;\r\n    }\r\n    if (this.touches.size > 2) return;\r\n    const t = { id: e.pointerId, x: e.clientX, y: e.clientY, dragging: false, done: false };\r\n    t.timer = setTimeout(() => {\r\n      // Long press: right click at the start point.\r\n      t.done = true;\r\n      this.mouseAt(WM.MOUSEMOVE, t.x, t.y, 0);\r\n      this.mouseAt(WM.RBUTTONDOWN, t.x, t.y, MK.RBUTTON);\r\n      this.mouseAt(WM.RBUTTONUP, t.x, t.y, 0);\r\n      if (navigator.vibrate) navigator.vibrate(15);\r\n    }, LONG_PRESS_MS);\r\n    this.touch = t;\r\n  }\r\n\r\n  touchMove(e) {\r\n    if (!this.touches.has(e.pointerId)) return;\r\n    this.touches.set(e.pointerId, { x: e.clientX, y: e.clientY });\r\n    if (this.pinch && this.touches.size === 2) {\r\n      const [a, b] = [...this.touches.values()];\r\n      const mid = { x: (a.x + b.x) / 2, y: (a.y + b.y) / 2 };\r\n      this.stage.scrollLeft -= mid.x - this.pinch.mid.x;\r\n      this.stage.scrollTop -= mid.y - this.pinch.mid.y;\r\n      this.pinch.mid = mid;\r\n      this.setZoom(this.pinch.zoom * Math.hypot(a.x - b.x, a.y - b.y) / this.pinch.dist, mid);\r\n      return;\r\n    }\r\n    const t = this.touch;\r\n    if (!t || t.id !== e.pointerId || t.done) return;\r\n    if (!t.dragging && Math.hypot(e.clientX - t.x, e.clientY - t.y) > TAP_SLOP_PX) {\r\n      clearTimeout(t.timer);\r\n      t.dragging = true;\r\n      this.mouseAt(WM.MOUSEMOVE, t.x, t.y, 0);\r\n      this.mouseAt(WM.LBUTTONDOWN, t.x, t.y, MK.LBUTTON);\r\n    }\r\n    if (t.dragging) this.mouseAt(WM.MOUSEMOVE, e.clientX, e.clientY, MK.LBUTTON);\r\n  }\r\n\r\n  touchUp(e) {\r\n    this.touches.delete(e.pointerId);\r\n    if (this.pinch) {\r\n      if (this.touches.size < 2) this.pinch = null;\r\n      return;\r\n    }\r\n    const t = this.touch;\r\n    if (!t || t.id !== e.pointerId) return;\r\n    clearTimeout(t.timer);\r\n    this.touch = null;\r\n    if (t.done) return;\r\n    if (!t.dragging) {\r\n      // Tap: a complete click at the touch point.\r\n      this.mouseAt(WM.MOUSEMOVE, t.x, t.y, 0);\r\n      this.mouseAt(WM.LBUTTONDOWN, t.x, t.y, MK.LBUTTON);\r\n    }\r\n    this.mouseAt(WM.LBUTTONUP, e.clientX, e.clientY, 0);\r\n    this.canvas.focus({ preventScroll: true });\r\n  }\r\n\r\n  cancelTouch() {\r\n    const t = this.touch;\r\n    if (!t) return;\r\n    clearTimeout(t.timer);\r\n    // A drag that turns into a pinch is released where it is.\r\n    if (t.dragging) this.mouseAt(WM.LBUTTONUP, t.x, t.y, 0);\r\n    this.touch = null;\r\n  }\r\n\r\n  // --- keyboard ----------------------------------------------------------------------\r\n\r\n  keyDown(e) {\r\n    this.hideTip(true);\r\n    if (this.split && e.code === 'Escape') { e.preventDefault(); this.splitEnd(true); return; }\r\n    const vk = VK[e.code];\r\n    if (vk) {\r\n      e.preventDefault();\r\n      this.send(`k ${WM.KEYDOWN} ${vk[0]} ${keyLParam(vk[1], false)}`);\r\n    } else if (e.key.length === 1 && !e.altKey && !e.metaKey) {\r\n      e.preventDefault();\r\n      if (e.ctrlKey) {\r\n        // Ctrl+letter shortcuts: control characters 1..26 are what Windows sends as WM_CHAR.\r\n        const code = e.key.toUpperCase().charCodeAt(0);\r\n        if (code >= 65 && code <= 90) this.send(`k ${WM.CHAR} ${code - 64} 1`);\r\n      } else {\r\n        this.send(`k ${WM.CHAR} ${e.key.charCodeAt(0)} 1`);\r\n      }\r\n    }\r\n  }\r\n\r\n  keyUp(e) {\r\n    const vk = VK[e.code];\r\n    if (vk) {\r\n      e.preventDefault();\r\n      this.send(`k ${WM.KEYUP} ${vk[0]} ${keyLParam(vk[1], true)}`);\r\n    }\r\n  }\r\n\r\n  // On-screen keyboard (touch devices): a hidden input collects what is typed.\r\n  // Soft keyboards often report key 'Unidentified' (keyCode 229), so text comes\r\n  // from input events and only named keys from keydown.\r\n  bindKeyboard() {\r\n    const k = this.kbd;\r\n    document.getElementById('kbd-btn').addEventListener('click', () => {\r\n      k.value = '';\r\n      k.focus();\r\n    });\r\n    k.addEventListener('keydown', (e) => {\r\n      if (VK[e.code]) this.keyDown(e);\r\n    });\r\n    k.addEventListener('keyup', (e) => {\r\n      if (VK[e.code]) this.keyUp(e);\r\n    });\r\n    k.addEventListener('beforeinput', (e) => {\r\n      e.preventDefault();\r\n      if (e.inputType === 'deleteContentBackward') {\r\n        this.send(`k ${WM.KEYDOWN} 8 ${keyLParam(0, false)}`);\r\n        this.send(`k ${WM.KEYUP} 8 ${keyLParam(0, true)}`);\r\n      } else if (e.inputType === 'insertLineBreak' || e.inputType === 'insertParagraph') {\r\n        this.send(`k ${WM.KEYDOWN} 13 ${keyLParam(0, false)}`);\r\n        this.send(`k ${WM.KEYUP} 13 ${keyLParam(0, true)}`);\r\n      } else if (typeof e.data === 'string') {\r\n        for (const ch of e.data) this.send(`k ${WM.CHAR} ${ch.codePointAt(0)} 1`);\r\n      }\r\n    });\r\n  }\r\n\r\n  // --- status ------------------------------------------------------------------------\r\n\r\n  setStatus(state, text) {\r\n    document.body.dataset.state = state;\r\n    this.statusEl.textContent = text;\r\n  }\r\n\r\n  toast(text) {\r\n    const el = document.getElementById('toast');\r\n    el.textContent = text;\r\n    el.classList.add('show');\r\n    clearTimeout(this.toastTimer);\r\n    this.toastTimer = setTimeout(() => el.classList.remove('show'), 1800);\r\n  }\r\n\r\n  showStats() {\r\n    const secs = (performance.now() - this.stats.since) / 1000;\r\n    this.statsEl.textContent =\r\n      `${(this.stats.frames / secs).toFixed(0)} fps | ${(this.stats.bytes / 1024 / secs).toFixed(0)} KiB/s`;\r\n    this.stats = { frames: 0, bytes: 0, since: performance.now() };\r\n  }\r\n}\r\n\r\nnew RemoteViClient();\r\n</script>\r\n</body>\r\n</html>\r\n"
  "error out" <- "error in"
